vi "[ex ce] History Speed (CE & DBL scalar).vi"() -> ()   [LabVIEW 2021]
doc: "<B>Run speed example</B>\n\nThe VI demonstrates how a variable history affects execution speed.\n\n::: CalcExpress Toolkit :::\nCopyright (c) 2000-2026 Konstantin Shifershteyn. All rights reserved."
panel:
  out "Historic values":dbl[](array[numeric]) format="%#_9g"
  in  "reverse order":bool=TRUE caption="Read history in reversed order"
  in  "number of iterations":i32=100000
  out "read history, ms":u32
  out "speed ratio":dbl format="%.2f"
  out "with history, ms":u32
  out "without history, ms":u32
  in  "history length":i32=10000
  in  "expression":string="x += 1;"
  # "execution time"
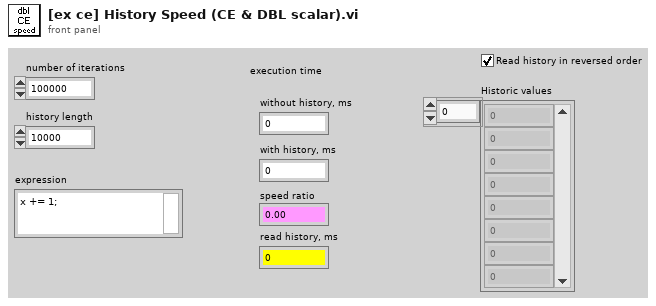
[diagram p1: front panel]
types:
  T1 = enum16{"create", "destroy", "set value", "get value"}
  T2 = enum32{"nop", "create", "destroy", "reset", "get info", "config"}
  T3 = typedef "VarMan Variable Context Handle.ctl" = i32
  T4 = typedef "CalcExpress Instance RefNum.ctl" = refnum<k1>
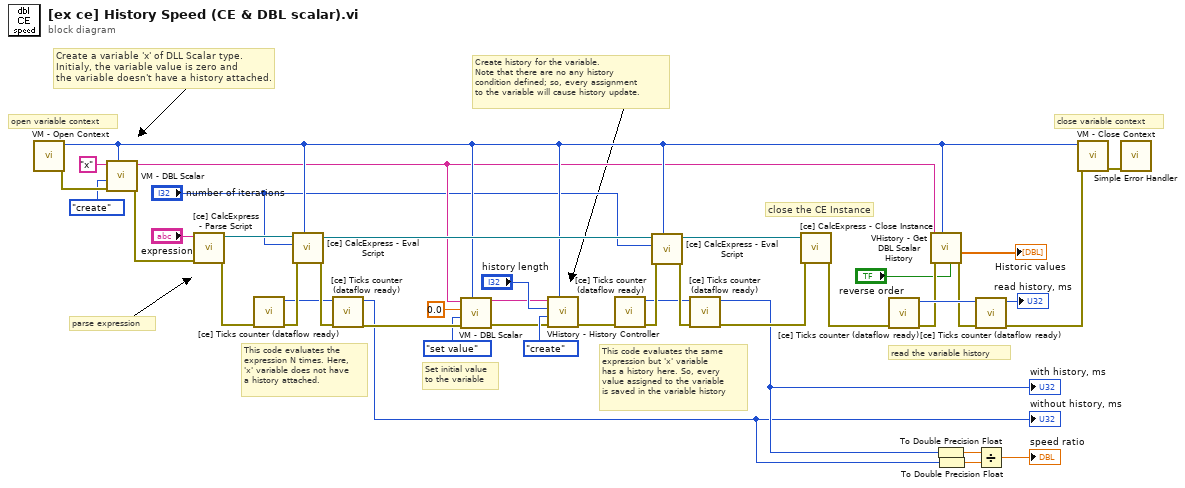
[diagram p0: block diagram]
diagram:
  # "Create history for the variable.\nNote that there are no any history\ncondition defined; so, every assignment\nto the variable will cause history update."
  # "Set initial value\nto the variable"
  # "This code evaluates the same\nexpression but 'x' variable\nhas a history here. So, every\nvalue assigned to the variable\nis saved in the variable history"
  # "This code evaluates the\nexpression N times. Here,\n'x' variable does not have\na history attached."
  # "Create a variable 'x' of DLL Scalar type.\nInitialy, the variable value is zero and\nthe variable doesn't have a history attached."
  # "close the CE Instance"
  # "close variable context"
  # "read the variable history"
  # "parse expression"
  # "open variable context"
  n1 = call "VM - Open Context.vi"() -> ("error out"=w39:errorcluster, "VC Handle out"=w12:T3)  [unwired: 9 in, 1 out]
  n2 = call "VM - DBL Scalar.vi"("VC Handle"=w12, "error in"=w39, "cmd"=T1."create", "name_spec"="x" ("name")) -> ("error out"=w25:errorcluster, "dup name_spec"=w11:string)  [unwired: 2 in, 4 out]
  n3 = call "[ce] CalcExpress - Parse Script.vi"("error in"=w25, "expression"="expression") -> ("error out"=w35:errorcluster, "CE InstanceRef"=w28:T4)  [unwired: 4 in, 2 out]
  n4 = call "[ce] Ticks counter (dataflow ready).vi"("error in"=w35) -> ("error out"=w34:errorcluster, "ticks (current-input)"=w24:u32)  [unwired: 4 in, 3 out]
  n5 = call "[ce] CalcExpress - Eval Script.vi"("VC Handle"=w12, "error in"=w34, "repeat (1)"="number of iterations", "CE InstanceRef"=w28) -> ("error out"=w33:errorcluster, "dup CE InstanceRef"=w29:T4)  [unwired: 1 in, 3 out]
  n6 = call "[ce] Ticks counter (dataflow ready).vi"("error in"=w33, "ticks in"=w24) -> ("error out"=w13:errorcluster, "ticks (current-input)"=w6:u32)  [unwired: 3 in, 3 out]
  "without history, ms" <- w6
  n7 = call "VM - DBL Scalar.vi"("VC Handle"=w12, "error in"=w13, "cmd"=T1."set value", "value in"=0.0, "name_spec"=w11) -> ("error out"=w14:errorcluster, "dup name_spec"=w15:string)  [unwired: 1 in, 4 out]
  n8 = call "VHistory - History Controller.vi"("VC Handle"=w12, "error in"=w14, "cmd (nop:default)"=T2."create", "history length"="history length", "name_spec"=w15) -> ("error out"=w30:errorcluster)  [unwired: 3 in, 3 out]
  n9 = call "[ce] Ticks counter (dataflow ready).vi"("error in"=w30) -> ("error out"=w31:errorcluster, "ticks (current-input)"=w23:u32)  [unwired: 4 in, 3 out]
  n10 = call "[ce] CalcExpress - Eval Script.vi"("VC Handle"=w12, "error in"=w31, "repeat (1)"="number of iterations", "CE InstanceRef"=w29) -> ("error out"=w32:errorcluster, "dup CE InstanceRef"=w27:T4)  [unwired: 1 in, 3 out]
  n11 = call "[ce] Ticks counter (dataflow ready).vi"("error in"=w32, "ticks in"=w23) -> ("error out"=w26:errorcluster, "ticks (current-input)"=w7:u32)  [unwired: 3 in, 3 out]
  "with history, ms" <- w7
  n12 = call "[ce] CalcExpress - Close Instance.vi"("error in"=w26, "CE InstanceRef"=w27) -> ("error out"=w20:errorcluster)  [unwired: 5 in, 2 out]
  n13 = call "[ce] Ticks counter (dataflow ready).vi"("error in"=w20) -> ("error out"=w19:errorcluster, "ticks (current-input)"=w21:u32)  [unwired: 4 in, 3 out]
  n14 = call "VHistory - Get DBL Scalar History.vi"("reverse order (T)"="reverse order", "VC Handle"=w12, "error in"=w19, "name_spec"=w11) -> ("error out"=w18:errorcluster, "history"=→"Historic values":dbl[])  [unwired: 3 in, 3 out]
  n15 = To Double Precision Float(number=w7) -> (double precision float=w2:dbl)
  n16 = To Double Precision Float(number=w6) -> (double precision float=w1:dbl)
  n17 = call "[ce] Ticks counter (dataflow ready).vi"("error in"=w18, "ticks in"=w21) -> ("error out"=w17:errorcluster, "ticks (current-input)"=→"read history, ms":u32)  [unwired: 3 in, 3 out]
  n18 = Divide(x=w2, y=w1) -> (x/y=→"speed ratio":dbl)
  n19 = call "VM - Close Context.vi"("error in"=w17, "VC Handle"=w12) -> ("error out"=w8:errorcluster)  [unwired: 8 in, 1 out]
  n20 = call <vilib>:"Simple Error Handler.vi"("error in (no error)"=w8) -> ()  [unwired: 4 in, 5 out]
